vi "lidar_dinamic_roi_set.vi"(11 "cmd":dbl) -> (0 "Z13_Half":dbl, 1 "Z13_Ctr":dbl, 2 "E_Half":dbl, 3 "Z2_Half":dbl, 5 "Z2_Ctr":dbl, 7 "E_Ctr":dbl)   [LabVIEW 2024]
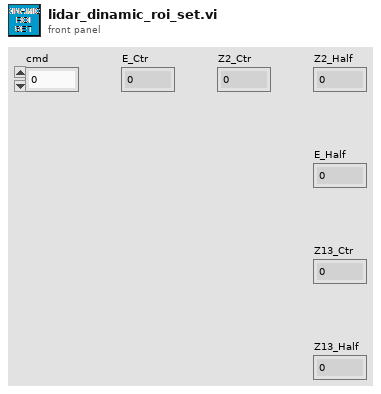
[diagram p1: front panel]
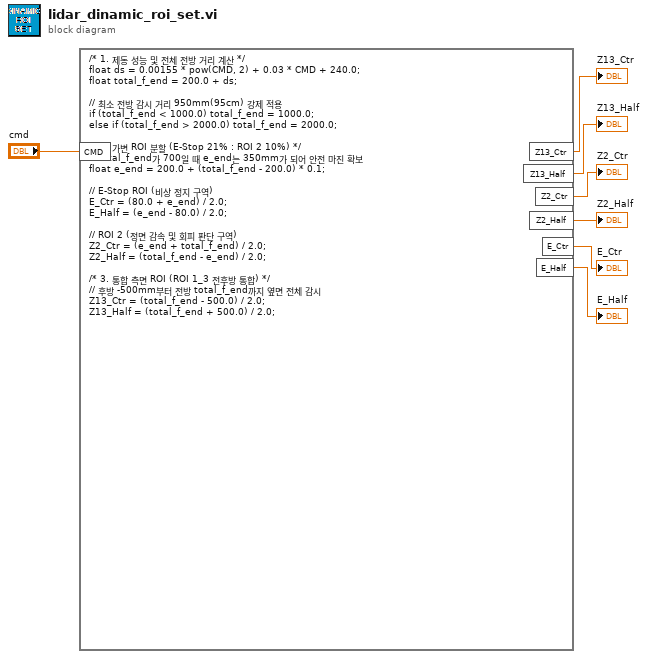
[diagram p0: block diagram]
diagram:
  n1 = formula code="/* 1. 제동 성능 및 전체 전방 거리 계산 */\nfloat ds = 0.00155 * pow(CMD, 2) + 0.03 * CMD + 240.0;\nfloat total_f_end = 200.0 + ds;\n\n// 최소 전방 감시 거리 950mm(95cm) 강제 적용\nif (total_f_end < 1000.0) total_f_end = 1000.0;\nelse if (total_f_end > 2000.0) total_f_end = 2000.0;\n\n/* 2. 가변 ROI 분할 (E-Stop 21% : ROI 2 10%) */\n// total_f_end가 700일 때 e_end는 350mm가 되어 안전 마진 확보\nfloat e_end = 200.0 + (total_f_end - 200.0) * 0.1;\n\n// E-Stop ROI (비상 정지 구역)\nE_Ctr = (80.0 + e_end) / 2.0;\nE_Half = (e_end - 80.0) / 2.0;\n\n// ROI 2 (정면 감속 및 회피 판단 구역)\nZ2_Ctr = (e_end + total_f_end) / 2.0;\nZ2_Half = (total_f_end - e_end) / 2.0;\n\n/* 3. 통합 측면 ROI (ROI 1_3 전후방 통합) */\n// 후방 -500mm부터 전방 total_f_end까지 옆면 전체 감시\nZ13_Ctr = (total_f_end - 500.0) / 2.0;\nZ13_Half = (total_f_end + 500.0) / 2.0;"("CMD"="cmd") -> ("Z13_Ctr"=→"Z13_Ctr":dbl, "Z13_Half"=→"Z13_Half":dbl, "Z2_Ctr"=→"Z2_Ctr":dbl, "Z2_Half"=→"Z2_Half":dbl, "E_Ctr"=→"E_Ctr":dbl, "E_Half"=→"E_Half":dbl)
